vi "configuration UI.vi"() -> ()   [LabVIEW 2013, in "EthernetIP editor node.lvclass"]
uses:
  EthernetIP editor node.lvclass
  <vilib>/NI/Configuration Framework/Node/NodeRef.ctl
  <vilib>/NI/Configuration Framework/Node/NISE_CEF_Node.lvclass
  <vilib>/NI/AMC/Message Queue.ctl
  <vilib>/NI/AMC/Message.ctl
  <vilib>/NI/Tools/Keyed Array/KeyedArray.ctl
  <vilib>/NI/Configuration Framework/Node/UserEventRef.ctl
  <vilib>/NI/Configuration Framework/Controls/EventCluster.ctl
  <vilib>/NI/DCAF UI Toolkit/Controls/Configure.ctl
  <vilib>/NI/DCAF UI Toolkit/Controls/Add.ctl
  <vilib>/NI/DCAF UI Toolkit/Controls/Remove.ctl
  configuration/EthernetIP configuration.lvclass
  EthernetIP editor node.lvclass/EthernetIP editor node.ctl
  <vilib>/NI/Configuration Framework/serializable configuration/NISE_CEF_serializable configuration.lvclass/NISE_CEF_serializable configuration.ctl
  <vilib>/NI/DCAF/Tag Editor Core/Configuration Editor/Classes/Module editor node/Read Module Configuration.vi
  <vilib>/Utility/LVClass/Get LV Class Name.vi
  <vilib>/NI/Configuration Framework/error generator/NISE_error generator.vi
  <vilib>/NI/Tag Bus Module Framework/module configuration/TBM module configuration.lvclass
  <vilib>/NI/Module Execution Interface/Engine Configuration/engine configuration.lvclass
  <vilib>/NI/Configuration Framework/NISE_CEF_TreeControl.lvlib
  <vilib>/NI/DCAF/Tag Editor Core/Configuration Editor/Classes/Module editor node/module editor node.lvclass
  <vilib>/NI/DCAF/Tag Editor Core/Configuration Editor/Classes/Engine Parent/Engine Parent Editor Node.lvclass
  <vilib>/NI/Configuration Framework/serializable configuration/NISE_CEF_serializable configuration.lvclass
  <vilib>/NI/Tools/Keyed Array/Tools_KeyedArray.lvlib
  <vilib>/NI/AMC/AMC.lvlib
  <vilib>/NI/DCAF UI Toolkit/Controls/DCAF UI Elements.lvlib
panel:
  in  "Top Level Tab Control":enum32{"Assemblies", "Channels"}(tab)
  in  "assemblies":i32(listbox)
  in  "Add Assembly":T1
  in  "Remove Assembly":T2
  in  "Configure Assembly":T3
  in  "create ch from asm":bool
  in  "settings":T3
  in  "channel":i32(listbox)
  in  "Add Button":T1
  in  "Remove Button":T2
  in  "user event":T4
  in  "main queue":T5
  in  "node ref":T6
  # "Assembly"
  # "Channel"
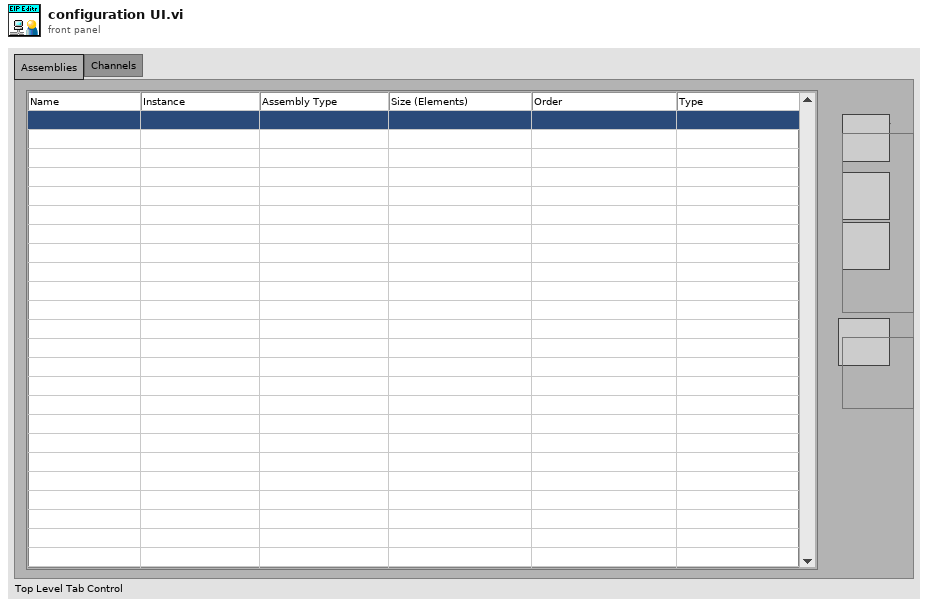
[diagram p1: front panel]
types:
  T1 = typedef "DCAF UI Elements.lvlib/Add.ctl" = bool
  T2 = typedef "DCAF UI Elements.lvlib/Remove.ctl" = bool
  T3 = typedef "DCAF UI Elements.lvlib/Configure.ctl" = bool
  T4 = typedef "NISE_CEF_Node.lvclass/UserEventRef.ctl" = refnum<user-event>
  T5 = typedef "AMC.lvlib/Message Queue.ctl" = refnum<queue>
  T6 = typedef "NISE_CEF_Node.lvclass/NodeRef.ctl" = refnum<data-value>
  T7 = typedef "NISE_CEF_TreeControl.lvlib/EventCluster.ctl" = cluster{"command":string, "data":string}
  T8 = typedef "EthernetIP configuration.lvclass/assembly definition.ctl" = cluster{"name":string, "Instance ID":u32, "Type":T9, "Size (elements)":u32, "big endian?":bool, "data type":T10}
  T9 = typedef "EthernetIP configuration.lvclass/assembly type.ctl" = enum32{"Producing", "Consuming"}
  T10 = typedef "tag bus.lvlib/tag descriptor.lvclass/Data Type.ctl" = enum16{"Double", "Single", "I64", "I32", "I16", "I8", "U64", "U32", "U16", "U8", "Boolean", "String", "Array of Double", "Array of Single", "Array of I64", "Array of I32", "Array of I16", "Array of I8", "Array of U64", "Array of U32", "Array of U16", "Array of U8", "Array of Boolean", "Array of String"}
  T11 = typedef "EthernetIP editor node.lvclass/table line.ctl" = cluster{"eip channels":refnum<class "EthernetIP Channel.lvclass">, "tag name":string}
  T12 = typedef "LVPoint32TypeDef.ctl" = cluster{"Horizontal":i32, "Vertical":i32}
  T13 = typedef "LVRowAndColumnTypeDef.ctl" = cluster{"Row":i32, "Column":i32}
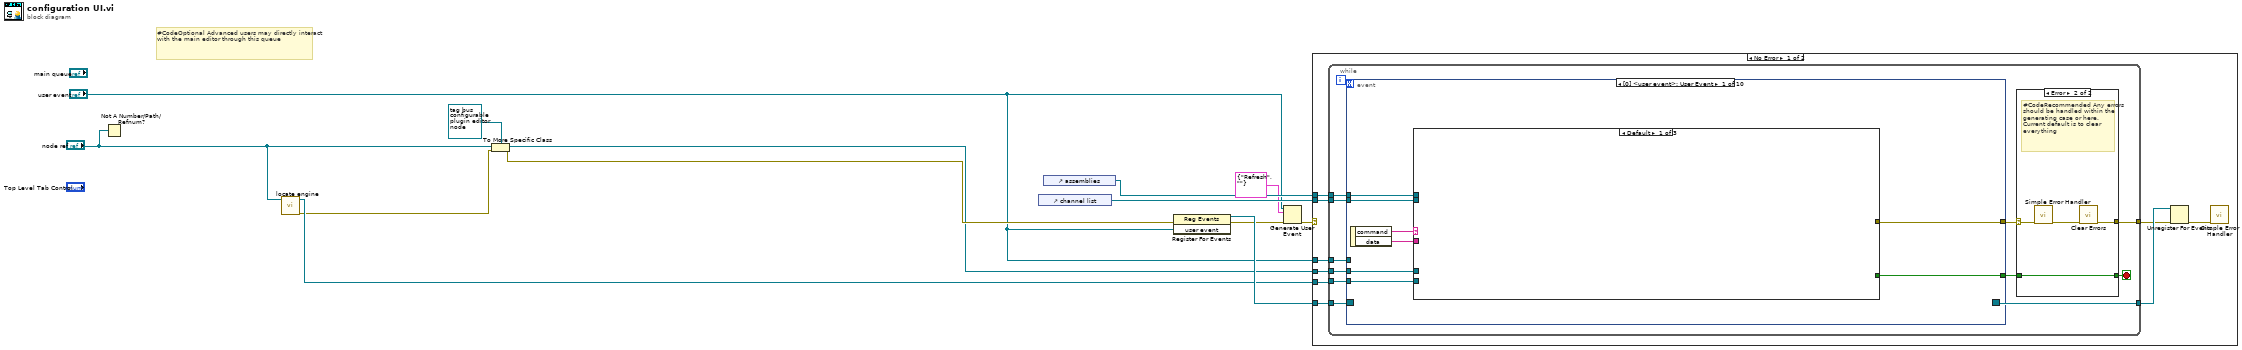
[diagram p0: block diagram]
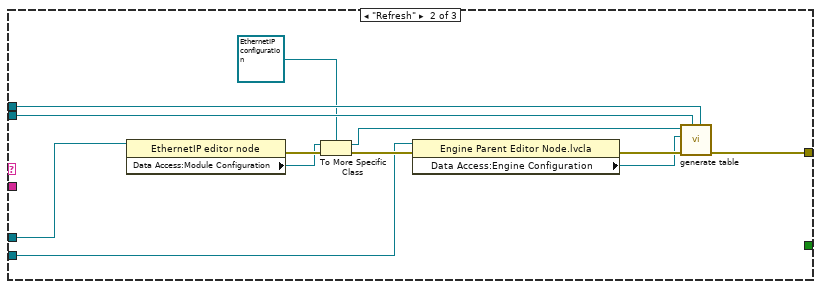
[diagram p3: hidden frame]
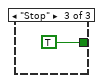
[diagram p4: hidden frame]
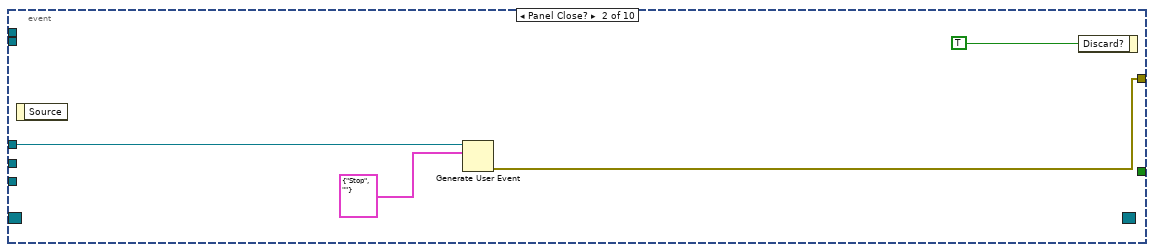
[diagram p5: hidden frame]
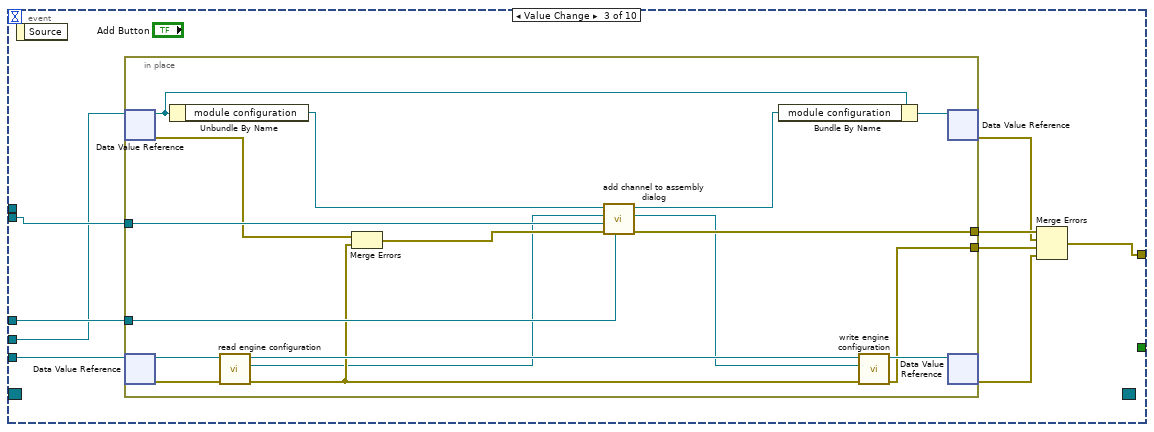
[diagram p6: hidden frame]
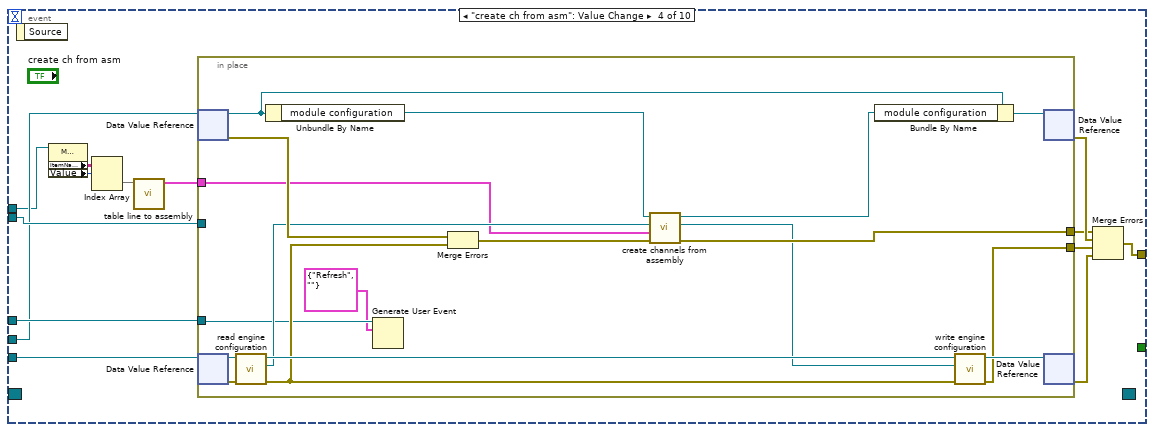
[diagram p7: hidden frame]
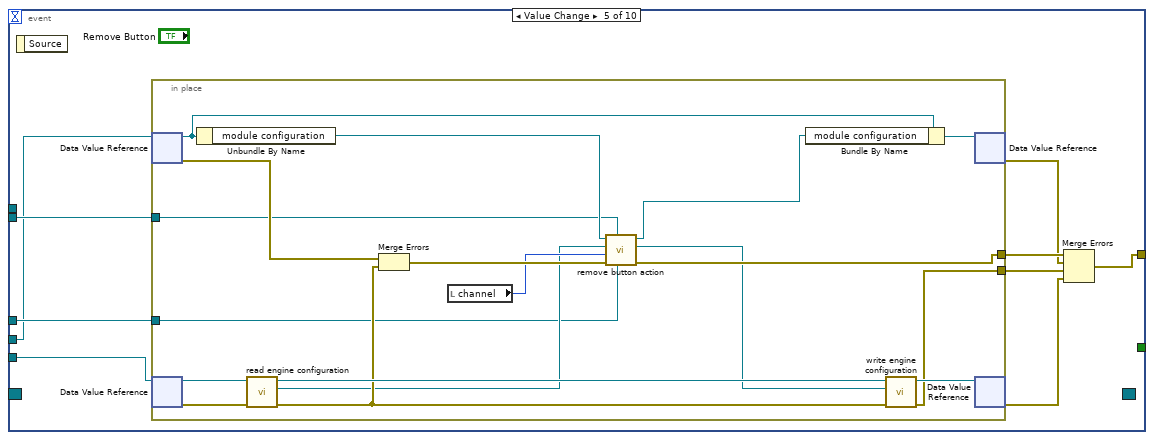
[diagram p8: hidden frame]
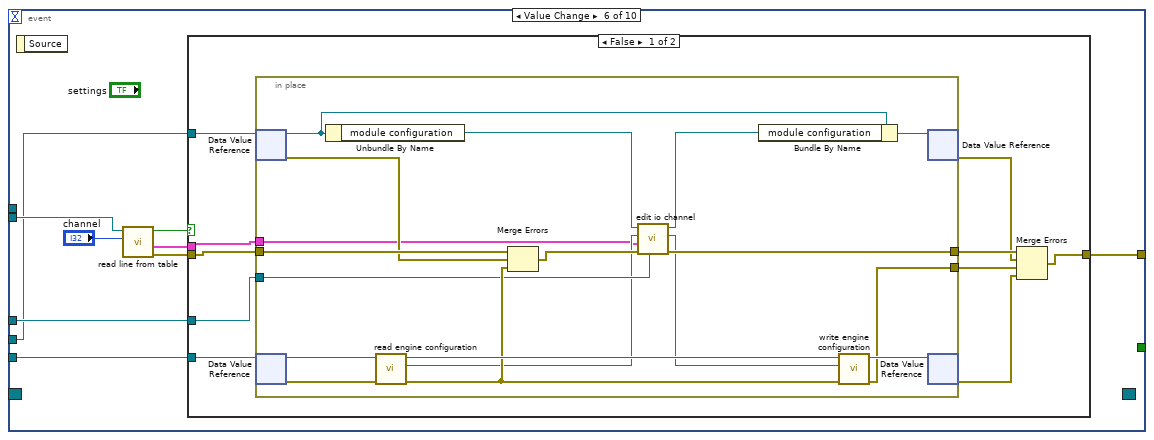
[diagram p9: hidden frame]
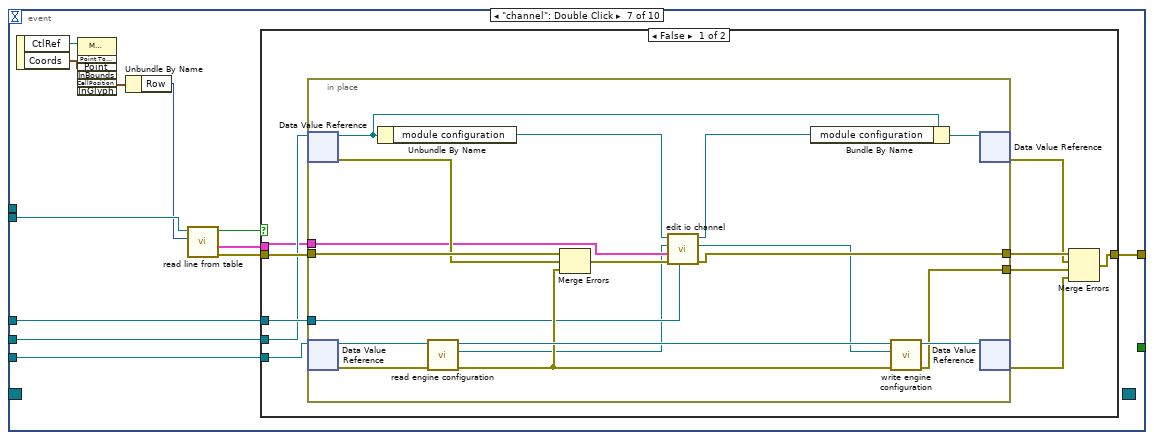
[diagram p11: hidden frame]
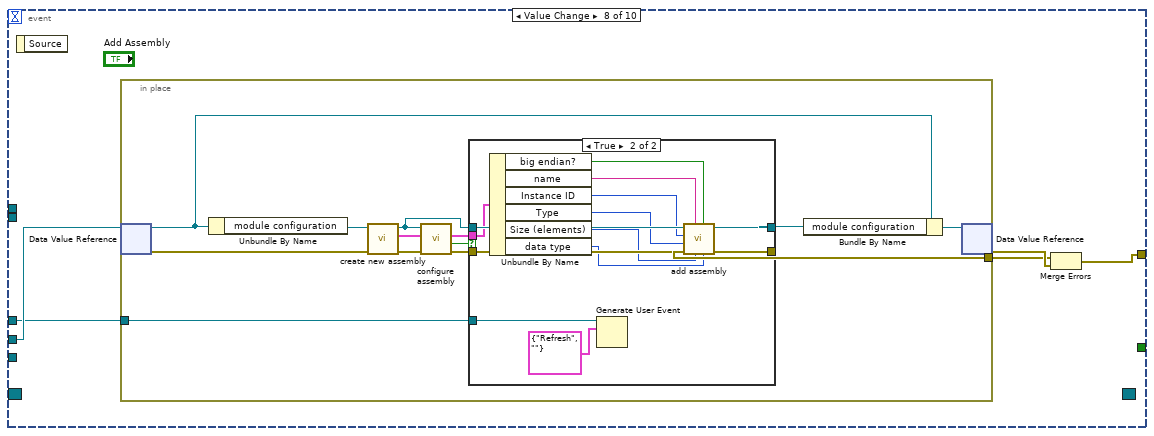
[diagram p13: hidden frame]
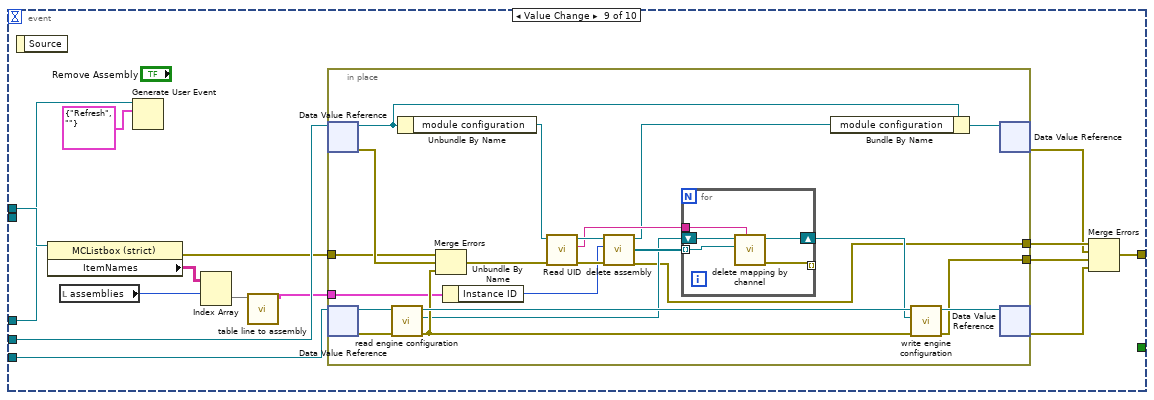
[diagram p15: hidden frame]
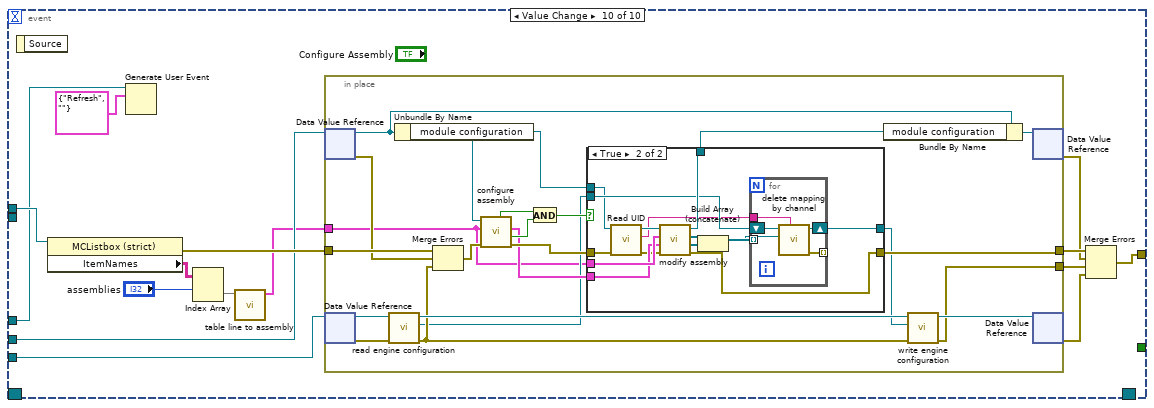
[diagram p16: hidden frame]
diagram:
  # "#CodeOptional Advanced users may directly interact with the main editor through this queue"
  n1 = Not A Number/Path/Refnum?(number/path/refnum="node ref") -> ()  [unwired: 1 out]
  n2 = call <vilib>:"locate engine.vi"("component"="node ref") -> ("error out"=w1:errorcluster, "engine"=w2:refnum<data-value>)  [unwired: 9 in]
  n3 = To More Specific Class(target class=refnum<data-value> refnum ("data value reference"), reference="node ref", error in=w1) -> (specific class reference=w10:refnum<data-value>, error out=w12:errorcluster)
  n4 = control-ref of="channel list"() -> (w9:refnum<vi>)
  n5 = control-ref of="assemblies"() -> (w8:refnum<vi>)
  n6 = register-events(error in=w12, "user event") -> (reference out=w13:refnum<event-registration>, error out=w5:errorcluster)  [unwired: 1 in]
  n7 = Generate User Event(user event="user event", event data cluster=T7 {"command"="Refresh", "data"=""} ("event data"), error in=w5) -> (error out=w4:errorcluster)  [unwired: 1 in, 1 out]
  n8 = case shown="No Error" w4 {
    tunnel: w13 -> [w22 _]
    tunnel: w10 -> [w19 _]
    tunnel: w2 -> [w18 _]
    tunnel: w9 -> [w16 _]
    tunnel: w8 -> [w15 _]
    tunnel: "user event" -> [w14 _]
    frame No Error {
      n9 = while {
        tunnel: w22 -> [w33]
        tunnel: [w32] -> w21
        tunnel: w19 -> [w28]
        tunnel: w18 -> [w27]
        tunnel: w14 -> [w26]
        tunnel: w16 -> [w24]
        tunnel: w15 -> [w23]
        tunnel: [w29] -> w20
        stop <- w31 stop-if-true
        n10 = event shown="[0] <user event>: User Event" {
          selector: w33 -> [_ _ _ _ _ _ _ _ _ _]
          dyn-events: [_ _ _ _ _ _ _ _ _ _] -> w32
          timeout: _ -> [_ _ _ _ _ _ _ _ _ _]
          tunnel: [w47 _ _ _ _ _ _ _ _ _] -> w30
          tunnel: [w42 w61 w68 w100 w127 w158 w199 w232 w267 w308] -> w25
          tunnel: w28 -> [w45 _ w70 w102 w123 w150 w188 w231 w266 w305]
          tunnel: w27 -> [w44 _ w69 w101 w124 w151 w189 _ w264 w306]
          tunnel: w26 -> [_ w63 w71 w103 w125 w154 w196 w229 w272 w313]
          tunnel: w24 -> [w41 _ w72 w104 w126 w152 w195 _ _ _]
          tunnel: w23 -> [w40 _ _ w94 _ _ _ _ w276 w318]
          event User Event {
            n11 = event-data() -> ("command"=w46:string, "data"=w43:string)  [unwired: 1 in]
            n12 = case shown="Default" w46 {
              tunnel: [_ _ TRUE] -> w47
              tunnel: w45 -> [_ w54 _]
              tunnel: w44 -> [_ w49 _]
              tunnel: w43 -> [_ _ _]
              tunnel: [_ w59 _] -> w42
              tunnel: w41 -> [_ w58 _]
              tunnel: w40 -> [_ w57 _]
              frame Default {
              }
              frame "Refresh" {
                n13 = property class="EthernetIP editor node"(reference=w54) -> (error out=w55:errorcluster, "Data Access:Module Configuration"=w52:refnum<class "TBM module configuration.lvclass">)  [unwired: 1 in, 1 out]
                n14 = To More Specific Class(target class=refnum<class "EthernetIP configuration.lvclass"> refnum ("tag bus configurable plugin module configuration"), reference=w52, error in=w55) -> (specific class reference=w50:refnum<class "EthernetIP configuration.lvclass">, error out=w53:errorcluster)
                n15 = property class="Engine Parent Editor Node.lvcla"(reference=w49, error in=w53) -> (error out=w56:errorcluster, "Data Access:Engine Configuration"=w48:refnum<class "engine configuration.lvclass">)  [unwired: 1 out]
                n16 = call "generate table.vi"("assemblies"=w57, "table"=w58, "error in"=w56, "engine configuration in"=w48, "EthernetIP configuration in"=w50) -> ("error out"=w59:errorcluster)  [unwired: 6 in]
              }
              frame "Stop" {
              }
            }
          }
          event Panel Close? {
            n17 = event-data() -> ()  [unwired: 1 in, 1 out]
            n18 = Generate User Event(user event=w63, event data cluster=T7 {"command"="Stop", "data"=""} ("event data")) -> (error out=w61:errorcluster)  [unwired: 2 in, 1 out]
            n19 = event-data("Discard?"=TRUE) -> ()  [unwired: 1 in, 1 out]
          }
          event Value Change {
            n20 = event-data() -> ()  [unwired: 1 in, 1 out]
            n21 = in-place {
              in-place-border: [w90] -> w73
              in-place-border: w72 -> [w89]
              in-place-border: w71 -> [w88]
              in-place-border: [w80] -> w65
              n22 = in-place-dvr #1(w70) -> (w86:refnum<class "EthernetIP editor node.lvclass">, w82:errorcluster)
              n23 = in-place-dvr #2(w69) -> (w79:refnum<class "Engine Parent Editor Node.lvclass">, w78:errorcluster)
              n24 = Unbundle By Name(w86) -> ("module configuration"=w87:refnum<class "EthernetIP configuration.lvclass">)
              n25 = call <vilib>:"read engine configuration.vi"("error in"=w78, "Engine Parent Editor Node in"=w79) -> ("error out"=w76:errorcluster, "engine configuration"=w74:refnum<class "engine configuration.lvclass">, "Engine Parent Editor Node out"=w77:refnum<class "Engine Parent Editor Node.lvclass">)  [unwired: 7 in]
              n26 = Merge Errors(w82, w76) -> (w83:errorcluster)
              n27 = call "add channel to assembly dialog.vi"("user event"=w88, "error in"=w83, "channel list"=w89, "engine configuration in"=w74, "EthernetIP configuration in"=w87) -> ("error out"=w90:errorcluster, "engine configuration out"=w75:refnum<class "engine configuration.lvclass">, "EthernetIP configuration out"=w84:refnum<class "EthernetIP configuration.lvclass">)  [unwired: 4 in]
              n28 = Bundle By Name(cluster=w86, "module configuration"=w84) -> (w85:refnum<class "EthernetIP editor node.lvclass">)
              n29 = call <vilib>:"write engine configuration.vi"("error in"=w76, "engine configuration"=w75, "Engine Parent Editor Node in"=w77) -> ("error out"=w80:errorcluster, "Engine Parent Editor Node out"=w81:refnum<class "Engine Parent Editor Node.lvclass">)  [unwired: 7 in]
              n30 = in-place-dvr #1(w85) -> (w66:errorcluster)  [unwired: 1 out]
              n31 = in-place-dvr #2(w81) -> (w67:errorcluster)  [unwired: 1 out]
            }
            n32 = Merge Errors(w73, w66, w65, w67) -> (w68:errorcluster)
          }
          event "create ch from asm": Value Change {
            n33 = event-data() -> ()  [unwired: 1 in, 1 out]
            n34 = property class="MCListbox (strict)"(reference=w94) -> ("ItemNames"=w95:string[][], "Value"=w96:i32)  [unwired: 1 in, 2 out]
            n35 = Index Array(array=w95, index (row)=w96) -> (element=w93:string[])  [unwired: 1 in]
            n36 = call "table line to assembly.vi"("ItemNames"=w93) -> ("assembly definition"=w91:T8)  [unwired: 10 in]
            n37 = in-place {
              in-place-border: w104 -> [_]
              in-place-border: w103 -> [w106]
              in-place-border: [w118] -> w97
              in-place-border: [w113] -> w92
              in-place-border: w91 -> [w107]
              n38 = in-place-dvr #3(w102) -> (w122:refnum<class "EthernetIP editor node.lvclass">, w120:errorcluster)
              n39 = in-place-dvr #4(w101) -> (w117:refnum<class "Engine Parent Editor Node.lvclass">, w116:errorcluster)
              n40 = call <vilib>:"read engine configuration.vi"("error in"=w116, "Engine Parent Editor Node in"=w117) -> ("error out"=w114:errorcluster, "engine configuration"=w108:refnum<class "engine configuration.lvclass">, "Engine Parent Editor Node out"=w115:refnum<class "Engine Parent Editor Node.lvclass">)  [unwired: 7 in]
              n41 = Unbundle By Name(w122) -> ("module configuration"=w111:refnum<class "EthernetIP configuration.lvclass">)
              n42 = Generate User Event(user event=w106, event data cluster=T7 {"command"="Refresh", "data"=""} ("event data")) -> ()  [unwired: 2 in, 2 out]
              n43 = Merge Errors(w120, w114) -> (w112:errorcluster)
              n44 = call "create channels from assembly.vi"("error in"=w112, "assembly definition"=w107, "engine configuration in"=w108, "EthernetIP configuration in"=w111) -> ("error out"=w113:errorcluster, "engine configuration out"=w109:refnum<class "engine configuration.lvclass">, "EthernetIP configuration out"=w110:refnum<class "EthernetIP configuration.lvclass">)  [unwired: 5 in]
              n45 = Bundle By Name(cluster=w122, "module configuration"=w110) -> (w121:refnum<class "EthernetIP editor node.lvclass">)
              n46 = call <vilib>:"write engine configuration.vi"("error in"=w114, "engine configuration"=w109, "Engine Parent Editor Node in"=w115) -> ("error out"=w118:errorcluster, "Engine Parent Editor Node out"=w119:refnum<class "Engine Parent Editor Node.lvclass">)  [unwired: 7 in]
              n47 = in-place-dvr #3(w121) -> (w98:errorcluster)  [unwired: 1 out]
              n48 = in-place-dvr #4(w119) -> (w99:errorcluster)  [unwired: 1 out]
            }
            n49 = Merge Errors(w92, w98, w97, w99) -> (w100:errorcluster)
          }
          event Value Change {
            n50 = event-data() -> ()  [unwired: 1 in, 1 out]
            n51 = in-place {
              in-place-border: [w139] -> w131
              in-place-border: [w145] -> w128
              in-place-border: w126 -> [w133]
              in-place-border: w125 -> [w132]
              n52 = in-place-dvr #5(w123) -> (w149:refnum<class "EthernetIP editor node.lvclass">, w147:errorcluster)
              n53 = in-place-dvr #6(w124) -> (w144:refnum<class "Engine Parent Editor Node.lvclass">, w143:errorcluster)
              n54 = Unbundle By Name(w149) -> ("module configuration"=w137:refnum<class "EthernetIP configuration.lvclass">)
              n55 = call <vilib>:"read engine configuration.vi"("error in"=w143, "Engine Parent Editor Node in"=w144) -> ("error out"=w141:errorcluster, "engine configuration"=w135:refnum<class "engine configuration.lvclass">, "Engine Parent Editor Node out"=w142:refnum<class "Engine Parent Editor Node.lvclass">)  [unwired: 7 in]
              n56 = Merge Errors(w147, w141) -> (w140:errorcluster)
              n57 = local read "channel"() -> (w136:i32)
              n58 = call "remove button action.vi"("user event"=w132, "channel list"=w133, "error in"=w140, "channel"=w136, "engine configuration in"=w135, "EthernetIP configuration in"=w137) -> ("error out"=w139:errorcluster, "engine configuration out"=w134:refnum<class "engine configuration.lvclass">, "EthernetIP configuration out"=w138:refnum<class "EthernetIP configuration.lvclass">)  [unwired: 3 in]
              n59 = Bundle By Name(cluster=w149, "module configuration"=w138) -> (w148:refnum<class "EthernetIP editor node.lvclass">)
              n60 = call <vilib>:"write engine configuration.vi"("error in"=w141, "engine configuration"=w134, "Engine Parent Editor Node in"=w142) -> ("error out"=w145:errorcluster, "Engine Parent Editor Node out"=w146:refnum<class "Engine Parent Editor Node.lvclass">)  [unwired: 7 in]
              n61 = in-place-dvr #5(w148) -> (w129:errorcluster)  [unwired: 1 out]
              n62 = in-place-dvr #6(w146) -> (w130:errorcluster)  [unwired: 1 out]
            }
            n63 = Merge Errors(w131, w129, w128, w130) -> (w127:errorcluster)
          }
          event Value Change {
            n64 = event-data() -> ()  [unwired: 1 in, 1 out]
            n65 = call "read line from table.vi"("line number"="channel", "channels table"=w152) -> ("error out"=w157:errorcluster, "line"=w156:T11, "empty channel?"=w153:bool)  [unwired: 6 in, 1 out]
            n66 = case shown="False" w153 {
              tunnel: [w163 w187] -> w158
              tunnel: w157 -> [w164 w187]
              tunnel: w156 -> [w159 _]
              tunnel: w154 -> [w162 _]
              tunnel: w151 -> [w161 _]
              tunnel: w150 -> [w160 _]
              frame False {
                n67 = in-place {
                  in-place-border: [w175] -> w168
                  in-place-border: w164 -> [w186]
                  in-place-border: [w181] -> w165
                  in-place-border: w162 -> [w174]
                  in-place-border: w159 -> [w169]
                  n68 = in-place-dvr #7(w160) -> (w185:refnum<class "EthernetIP editor node.lvclass">, w183:errorcluster)
                  n69 = in-place-dvr #8(w161) -> (w180:refnum<class "Engine Parent Editor Node.lvclass">, w179:errorcluster)
                  n70 = Unbundle By Name(w185) -> ("module configuration"=w173:refnum<class "EthernetIP configuration.lvclass">)
                  n71 = call <vilib>:"read engine configuration.vi"("error in"=w179, "Engine Parent Editor Node in"=w180) -> ("error out"=w177:errorcluster, "engine configuration"=w170:refnum<class "engine configuration.lvclass">, "Engine Parent Editor Node out"=w178:refnum<class "Engine Parent Editor Node.lvclass">)  [unwired: 7 in]
                  n72 = Merge Errors(w186, w183, w177) -> (w176:errorcluster)
                  n73 = call "edit io channel.vi"("user event"=w174, "error in"=w176, "line"=w169, "engine configuration in"=w170, "EthernetIP configuration in"=w173) -> ("error out"=w175:errorcluster, "engine configuration out"=w171:refnum<class "engine configuration.lvclass">, "EthernetIP configuration out"=w172:refnum<class "EthernetIP configuration.lvclass">)  [unwired: 4 in]
                  n74 = Bundle By Name(cluster=w185, "module configuration"=w172) -> (w184:refnum<class "EthernetIP editor node.lvclass">)
                  n75 = call <vilib>:"write engine configuration.vi"("error in"=w177, "engine configuration"=w171, "Engine Parent Editor Node in"=w178) -> ("error out"=w181:errorcluster, "Engine Parent Editor Node out"=w182:refnum<class "Engine Parent Editor Node.lvclass">)  [unwired: 7 in]
                  n76 = in-place-dvr #7(w184) -> (w166:errorcluster)  [unwired: 1 out]
                  n77 = in-place-dvr #8(w182) -> (w167:errorcluster)  [unwired: 1 out]
                }
                n78 = Merge Errors(w168, w166, w165, w167) -> (w163:errorcluster)
              }
              frame True {
              }
            }
          }
          event "channel": Double Click {
            n79 = event-data() -> ("CtlRef"=w194:refnum<vi>, "Coords"=w193:T12)  [unwired: 1 in]
            n80 = invoke class="MCListbox (strict)" method="Point To Row Column"(reference=w194, "Point"=w193) -> ("CellPosition"=w192:T13)  [unwired: 5 in, 6 out]
            n81 = Unbundle By Name(w192) -> ("Row"=w191:i32)
            n82 = call "read line from table.vi"("line number"=w191, "channels table"=w195) -> ("error out"=w198:errorcluster, "line"=w197:T11, "empty channel?"=w190:bool)  [unwired: 6 in, 1 out]
            n83 = case shown="False" w190 {
              tunnel: [w205 w228] -> w199
              tunnel: w198 -> [w204 w228]
              tunnel: w197 -> [w200 _]
              tunnel: w196 -> [w203 _]
              tunnel: w189 -> [w202 _]
              tunnel: w188 -> [w201 _]
              frame False {
                n84 = in-place {
                  in-place-border: [w216] -> w209
                  in-place-border: w204 -> [w227]
                  in-place-border: [w222] -> w206
                  in-place-border: w203 -> [w215]
                  in-place-border: w200 -> [w214]
                  n85 = in-place-dvr #9(w201) -> (w226:refnum<class "EthernetIP editor node.lvclass">, w224:errorcluster)
                  n86 = in-place-dvr #10(w202) -> (w221:refnum<class "Engine Parent Editor Node.lvclass">, w220:errorcluster)
                  n87 = Unbundle By Name(w226) -> ("module configuration"=w213:refnum<class "EthernetIP configuration.lvclass">)
                  n88 = call <vilib>:"read engine configuration.vi"("error in"=w220, "Engine Parent Editor Node in"=w221) -> ("error out"=w218:errorcluster, "engine configuration"=w210:refnum<class "engine configuration.lvclass">, "Engine Parent Editor Node out"=w219:refnum<class "Engine Parent Editor Node.lvclass">)  [unwired: 7 in]
                  n89 = Merge Errors(w227, w224, w218) -> (w217:errorcluster)
                  n90 = call "edit io channel.vi"("user event"=w215, "error in"=w217, "line"=w214, "engine configuration in"=w210, "EthernetIP configuration in"=w213) -> ("error out"=w216:errorcluster, "engine configuration out"=w211:refnum<class "engine configuration.lvclass">, "EthernetIP configuration out"=w212:refnum<class "EthernetIP configuration.lvclass">)  [unwired: 4 in]
                  n91 = Bundle By Name(cluster=w226, "module configuration"=w212) -> (w225:refnum<class "EthernetIP editor node.lvclass">)
                  n92 = call <vilib>:"write engine configuration.vi"("error in"=w218, "engine configuration"=w211, "Engine Parent Editor Node in"=w219) -> ("error out"=w222:errorcluster, "Engine Parent Editor Node out"=w223:refnum<class "Engine Parent Editor Node.lvclass">)  [unwired: 7 in]
                  n93 = in-place-dvr #9(w225) -> (w207:errorcluster)  [unwired: 1 out]
                  n94 = in-place-dvr #10(w223) -> (w208:errorcluster)  [unwired: 1 out]
                }
                n95 = Merge Errors(w209, w207, w206, w208) -> (w205:errorcluster)
              }
              frame True {
              }
            }
          }
          event Value Change {
            n96 = event-data() -> ()  [unwired: 1 in, 1 out]
            n97 = in-place {
              in-place-border: [w235] -> w230
              in-place-border: w229 -> [w234]
              n98 = in-place-dvr #11(w231) -> (w246:refnum<class "EthernetIP editor node.lvclass">, w238:errorcluster)
              n99 = Unbundle By Name(w246) -> ("module configuration"=w237:refnum<class "EthernetIP configuration.lvclass">)
              n100 = call "create new assembly.vi"("error in (no error)"=w238, "EthernetIP configuration in"=w237) -> ("error out"=w241:errorcluster, "assembly definition out"=w239:T8, "EthernetIP configuration out"=w240:refnum<class "EthernetIP configuration.lvclass">)  [unwired: 7 in]
              n101 = call "configure assembly.vi"("error in"=w241, "assembly definition in"=w239, "EthernetIP configuration"=w240) -> ("error out"=w244:errorcluster, "success"=w242:bool, "assembly definition out"=w243:T8)  [unwired: 5 in, 1 out]
              n102 = case shown="True" w242 {
                tunnel: w244 -> [w247 w261]
                tunnel: [w247 w260] -> w235
                tunnel: [w248 w259] -> w236
                tunnel: w240 -> [w248 w258]
                tunnel: w243 -> [_ w257]
                tunnel: w234 -> [_ w250]
                frame False {
                }
                frame True {
                  n103 = Unbundle By Name(w257) -> ("big endian?"=w252:bool, "name"=w253:string, "Instance ID"=w254:u32, "Type"=w255:T9, "Size (elements)"=w256:u32, "data type"=w249:T10)
                  n104 = Generate User Event(user event=w250, event data cluster=T7 {"command"="Refresh", "data"=""} ("event data")) -> ()  [unwired: 2 in, 2 out]
                  n105 = call "add assembly.vi"("data type"=w249, "big endian?"=w252, "size (elements)"=w256, "name"=w253, "error in"=w261, "Type"=w255, "instance ID"=w254, "EthernetIP configuration in"=w258) -> ("error out"=w260:errorcluster, "EthernetIP configuration out"=w259:refnum<class "EthernetIP configuration.lvclass">)  [unwired: 2 in]
                }
              }
              n106 = Bundle By Name(cluster=w246, "module configuration"=w236) -> (w245:refnum<class "EthernetIP editor node.lvclass">)
              n107 = in-place-dvr #11(w245) -> (w233:errorcluster)  [unwired: 1 out]
            }
            n108 = Merge Errors(w230, w233) -> (w232:errorcluster)
          }
          event Value Change {
            n109 = event-data() -> ()  [unwired: 1 in, 1 out]
            n110 = property class="MCListbox (strict)"(reference=w276) -> (error out=w265:errorcluster, "ItemNames"=w275:string[][])  [unwired: 1 in, 1 out]
            n111 = local read "assemblies"() -> (w274:i32)
            n112 = Generate User Event(user event=w272, event data cluster=T7 {"command"="Refresh", "data"=""} ("event data")) -> ()  [unwired: 2 in, 2 out]
            n113 = Index Array(array=w275, index (row)=w274) -> (element=w263:string[])  [unwired: 1 in]
            n114 = call "table line to assembly.vi"("ItemNames"=w263) -> ("assembly definition"=w262:T8)  [unwired: 10 in]
            n115 = in-place {
              in-place-border: [w280] -> w271
              in-place-border: [w294] -> w268
              in-place-border: w262 -> [w278]
              in-place-border: w265 -> [w289]
              n116 = in-place-dvr #12(w266) -> (w298:refnum<class "EthernetIP editor node.lvclass">, w296:errorcluster)
              n117 = in-place-dvr #13(w264) -> (w293:refnum<class "Engine Parent Editor Node.lvclass">, w292:errorcluster)
              n118 = call <vilib>:"read engine configuration.vi"("error in"=w292, "Engine Parent Editor Node in"=w293) -> ("error out"=w290:errorcluster, "engine configuration"=w282:refnum<class "engine configuration.lvclass">, "Engine Parent Editor Node out"=w291:refnum<class "Engine Parent Editor Node.lvclass">)  [unwired: 7 in]
              n119 = Unbundle By Name(w298) -> ("module configuration"=w283:refnum<class "EthernetIP configuration.lvclass">)
              n120 = Merge Errors(w289, w296, w290) -> (w284:errorcluster)
              n121 = Unbundle By Name(w278) -> ("Instance ID"=w277:u32)
              n122 = call <vilib>:"Read UID.vi"("error in"=w284, "configuration in"=w283) -> ("error out"=w287:errorcluster, "instance id"=w285:string, "configuration out"=w286:refnum<class "EthernetIP configuration.lvclass">)  [unwired: 7 in]
              n123 = call "delete assembly.vi"("error in"=w287, "instance ID"=w277, "EthernetIP configuration in"=w286) -> ("error out"=w280:errorcluster, "invalidated channels"=w288:refnum<class "EthernetIP Channel.lvclass">[], "EthernetIP configuration out"=w279:refnum<class "EthernetIP configuration.lvclass">)  [unwired: 6 in]
              n124 = for {
                shift-right: [w303] -> w281
                shift-left: w282 -> [w302]
                tunnel: w288 -> [w301] mode=indexing
                tunnel: [w300] -> _ mode=indexing
                tunnel: w285 -> [w299]
                n125 = call <vilib>:"delete mapping by channel.vi"("owner ID"=w299, "channel"=w301, "engine configuration in"=w302) -> ("error out"=w300:errorcluster, "engine configuration out"=w303:refnum<class "engine configuration.lvclass">)  [unwired: 7 in]
              }
              n126 = Bundle By Name(cluster=w298, "module configuration"=w279) -> (w297:refnum<class "EthernetIP editor node.lvclass">)
              n127 = call <vilib>:"write engine configuration.vi"("error in"=w290, "engine configuration"=w281, "Engine Parent Editor Node in"=w291) -> ("error out"=w294:errorcluster, "Engine Parent Editor Node out"=w295:refnum<class "Engine Parent Editor Node.lvclass">)  [unwired: 7 in]
              n128 = in-place-dvr #12(w297) -> (w269:errorcluster)  [unwired: 1 out]
              n129 = in-place-dvr #13(w295) -> (w270:errorcluster)  [unwired: 1 out]
            }
            n130 = Merge Errors(w271, w269, w268, w270) -> (w267:errorcluster)
          }
          event Value Change {
            n131 = event-data() -> ()  [unwired: 1 in, 1 out]
            n132 = property class="MCListbox (strict)"(reference=w318) -> (error out=w307:errorcluster, "ItemNames"=w317:string[][])  [unwired: 1 in, 1 out]
            n133 = Generate User Event(user event=w313, event data cluster=T7 {"command"="Refresh", "data"=""} ("event data")) -> ()  [unwired: 2 in, 2 out]
            n134 = Index Array(array=w317, index (row)="assemblies") -> (element=w315:string[])  [unwired: 1 in]
            n135 = call "table line to assembly.vi"("ItemNames"=w315) -> ("assembly definition"=w304:T8)  [unwired: 10 in]
            n136 = in-place {
              in-place-border: [w325] -> w312
              in-place-border: w307 -> [w340]
              in-place-border: [w335] -> w309
              in-place-border: w304 -> [w319]
              n137 = in-place-dvr #14(w305) -> (w339:refnum<class "EthernetIP editor node.lvclass">, w337:errorcluster)
              n138 = in-place-dvr #15(w306) -> (w334:refnum<class "Engine Parent Editor Node.lvclass">, w333:errorcluster)
              n139 = call <vilib>:"read engine configuration.vi"("error in"=w333, "Engine Parent Editor Node in"=w334) -> ("error out"=w331:errorcluster, "engine configuration"=w320:refnum<class "engine configuration.lvclass">, "Engine Parent Editor Node out"=w332:refnum<class "Engine Parent Editor Node.lvclass">)  [unwired: 7 in]
              n140 = Unbundle By Name(w339) -> ("module configuration"=w321:refnum<class "EthernetIP configuration.lvclass">)
              n141 = Merge Errors(w340, w337, w331) -> (w322:errorcluster)
              n142 = call "configure assembly.vi"("error in"=w322, "assembly definition in"=w319, "EthernetIP configuration"=w321) -> ("error out"=w327:errorcluster, "success"=w330:bool, "assembly definition out"=w326:T8, "changed"=w329:bool)  [unwired: 5 in]
              n143 = And(x=w329, y=w330) -> (x .and. y?=w328:bool)
              n144 = case shown="True" w328 {
                tunnel: w327 -> [w343 w348]
                tunnel: [w343 w351] -> w325
                tunnel: w321 -> [w342 w344]
                tunnel: [w342 w357] -> w323
                tunnel: w319 -> [_ w356]
                tunnel: w326 -> [_ w355]
                tunnel: w320 -> [w341 w354]
                tunnel: [w341 w353] -> w324
                frame False {
                }
                frame True {
                  n145 = call <vilib>:"Read UID.vi"("error in"=w348, "configuration in"=w344) -> ("error out"=w347:errorcluster, "instance id"=w345:string, "configuration out"=w346:refnum<class "EthernetIP configuration.lvclass">)  [unwired: 7 in]
                  n146 = call "modify assembly.vi"("error in"=w347, "new"=w355, "original"=w356, "EthernetIP configuration in"=w346) -> ("error out"=w351:errorcluster, "channel type/dir changed"=w349:refnum<class "EthernetIP Channel.lvclass">[], "invalidated channels"=w352:refnum<class "EthernetIP Channel.lvclass">[], "EthernetIP configuration out"=w357:refnum<class "EthernetIP configuration.lvclass">)  [unwired: 4 in]
                  n147 = Build Array (concatenate)(w352, w349) -> (w350:refnum<class "EthernetIP Channel.lvclass">[])
                  n148 = for {
                    shift-right: [w362] -> w353
                    shift-left: w354 -> [w361]
                    tunnel: w350 -> [w360] mode=indexing
                    tunnel: [w359] -> _ mode=indexing
                    tunnel: w345 -> [w358]
                    n149 = call <vilib>:"delete mapping by channel.vi"("owner ID"=w358, "channel"=w360, "engine configuration in"=w361) -> ("error out"=w359:errorcluster, "engine configuration out"=w362:refnum<class "engine configuration.lvclass">)  [unwired: 7 in]
                  }
                }
              }
              n150 = Bundle By Name(cluster=w339, "module configuration"=w323) -> (w338:refnum<class "EthernetIP editor node.lvclass">)
              n151 = call <vilib>:"write engine configuration.vi"("error in"=w331, "engine configuration"=w324, "Engine Parent Editor Node in"=w332) -> ("error out"=w335:errorcluster, "Engine Parent Editor Node out"=w336:refnum<class "Engine Parent Editor Node.lvclass">)  [unwired: 7 in]
              n152 = in-place-dvr #14(w338) -> (w310:errorcluster)  [unwired: 1 out]
              n153 = in-place-dvr #15(w336) -> (w311:errorcluster)  [unwired: 1 out]
            }
            n154 = Merge Errors(w312, w310, w309, w311) -> (w308:errorcluster)
          }
        }
        n155 = case shown="Error" w25 {
          selector: w25 -> [w34 w38]
          tunnel: [w35 w39] -> w31
          tunnel: w30 -> [w35 w39]
          tunnel: [w34 w36] -> w29
          frame No Error {
          }
          frame Error {
            # "#CodeRecommended Any errors should be handled within the generating case or here. Current default is to clear everything"
            n156 = call <vilib>:"Simple Error Handler.vi"("error in (no error)"=w38) -> ("error out"=w37:errorcluster)  [unwired: 4 in, 4 out]
            n157 = call <vilib>:"Clear Errors.vi"("error in (no error)"=w37) -> ("error out"=w36:errorcluster)  [unwired: 6 in]
          }
        }
      }
      n158 = Unregister For Events(event registration refnum=w21, error in=w20) -> (error out=w17:errorcluster)
      n159 = call <vilib>:"Simple Error Handler.vi"("error in (no error)"=w17) -> ()  [unwired: 4 in, 5 out]
    }
    frame Error {
    }
  }
